vi "Open and Setup CAN Session.vi"(8 "error in":errorcluster, 11 "measurement configuration":T1 {"Baudrate" format="%x"; "FD Baudrate" format="%x"}) -> (0 "error out":errorcluster, 2 "session out":refnum<k21>)   [LabVIEW 2025, in "CAN-LIN Raw Bus Capture.lvclass"]
uses:
  CAN-LIN Raw Bus Capture.lvclass
  Measurement Configuration.ctl
  CAN-LIN Raw Bus Capture UI/Toggle.ctl
  <vilib>/xnet/xnet.llb/XNET Create Session (Frame Input Stream).vi
  CAN-LIN Raw Bus Capture.lvclass/CAN-LIN Raw Bus Capture.ctl
  <resource>/objmgr/xnet.rc
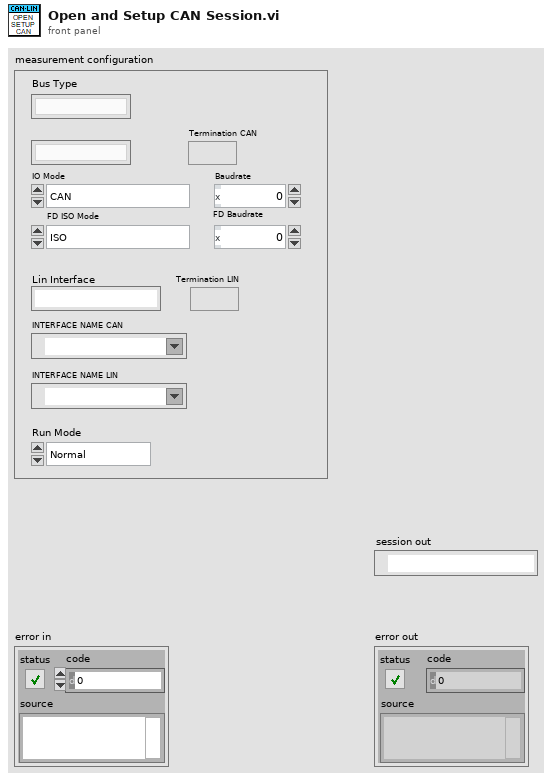
[diagram p1: front panel]
types:
  T1 = typedef "CAN-LIN Raw Bus Capture.lvclass/Measurement Configuration.ctl" = cluster{"Termination CAN":T2, "FD Baudrate":u32, "Baudrate":u32, "FD ISO Mode":enum32{"ISO", "Legacy ISO", "Non-ISO"}, "IO Mode":enum32{"CAN", "CAN FD", "CAN FD + BRS"}, "Termination LIN":T2, "Can Interface":string, "Lin Interface":string, "Bus Type":string, "INTERFACE NAME CAN":refnum<k21>, "INTERFACE NAME LIN":refnum<k21>, "Run Mode":enum32{"Normal", "Subordinate"}}
  T2 = typedef "Toggle.ctl" = bool
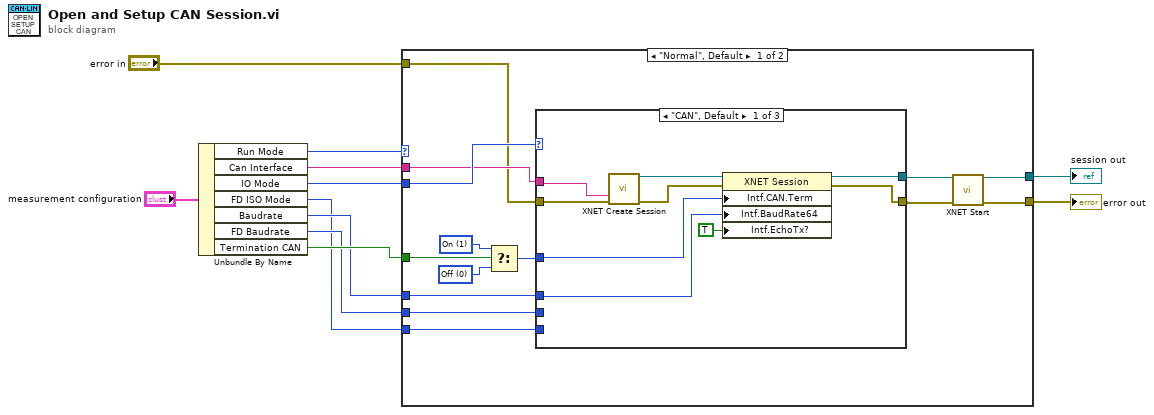
[diagram p0: block diagram]
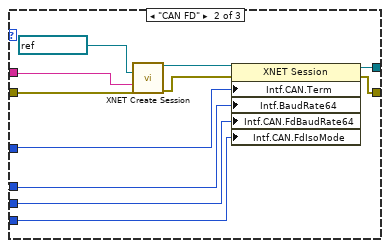
[diagram p2: hidden frame]
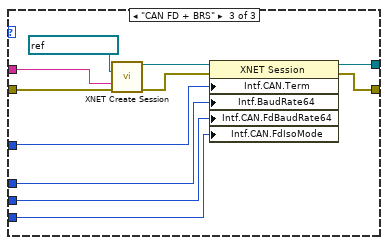
[diagram p3: hidden frame]
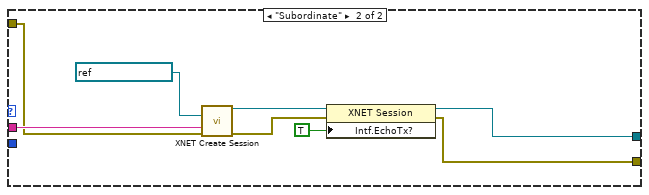
[diagram p4: hidden frame]
diagram:
  n1 = Unbundle By Name("measurement configuration") -> ("Run Mode"=w1:enum32{"Normal", "Subordinate"}, "Can Interface"=w6:string, "IO Mode"=w10:enum32{"CAN", "CAN FD", "CAN FD + BRS"}, "FD ISO Mode"=w7:enum32{"ISO", "Legacy ISO", "Non-ISO"}, "Baudrate"=w9:u32, "FD Baudrate"=w8:u32, "Termination CAN"=w11:T2)
  n2 = case shown="\"Normal\", Default" w1 {
    tunnel: w11 -> [w25 _]
    tunnel: w10 -> [w22 _]
    tunnel: w9 -> [w20 _]
    tunnel: w8 -> [w19 _]
    tunnel: w7 -> [w18 _]
    tunnel: w6 -> [w17 w61]
    tunnel: "error in" -> [w16 w57]
    tunnel: [w13 w58] -> w3
    tunnel: [w12 w59] -> w2
    frame "Normal", Default {
      w23 = u32 1 items=["Off", "On"] ("Interface:CAN:Termination")
      w24 = u32 0 items=["Off", "On"] ("Interface:CAN:Termination")
      n3 = Select(t=w23, s=w25, f=w24) -> (s? t:f=w21:u32)
      n4 = case shown="\"CAN\", Default" w22 {
        tunnel: [w32 w38 w53] -> w15
        tunnel: w17 -> [w29 w42 w49]
        tunnel: w16 -> [w31 w41 w48]
        tunnel: [w30 w37 w46] -> w14
        tunnel: w20 -> [w27 w40 w52]
        tunnel: w19 -> [_ w36 w51]
        tunnel: w18 -> [_ w39 w50]
        tunnel: w21 -> [w28 w35 w47]
        frame "CAN", Default {
          n5 = call-poly <vilib>:"XNET Create Session.vi"("interface"=w29, "error in (no error)"=w31) -> ("session out"=w34:refnum<k21>, "error out"=w33:errorcluster)  [unwired: 12 in]
          n6 = property class="XNET Session"(reference=w34, error in=w33, "Intf.CAN.Term"=w28, "Intf.BaudRate64"=w27, "Intf.EchoTx?"=TRUE ("Interface:Echo Transmit?")) -> (reference out=w32:refnum<k21>, error out=w30:errorcluster)
        }
        frame "CAN FD" {
          n7 = call-poly <vilib>:"XNET Create Session.vi"("cluster (:memory:)"=refnum<k21> ":can_fd:", "interface"=w42, "error in (no error)"=w41) -> ("session out"=w44:refnum<k21>, "error out"=w43:errorcluster)  [unwired: 11 in]
          n8 = property class="XNET Session"(reference=w44, error in=w43, "Intf.CAN.Term"=w35, "Intf.BaudRate64"=w40, "Intf.CAN.FdBaudRate64"=w36, "Intf.CAN.FdIsoMode"=w39) -> (reference out=w38:refnum<k21>, error out=w37:errorcluster)
        }
        frame "CAN FD + BRS" {
          n9 = call-poly <vilib>:"XNET Create Session.vi"("cluster (:memory:)"=refnum<k21> ":can_fd_brs:", "interface"=w49, "error in (no error)"=w48) -> ("session out"=w55:refnum<k21>, "error out"=w54:errorcluster)  [unwired: 11 in]
          n10 = property class="XNET Session"(reference=w55, error in=w54, "Intf.CAN.Term"=w47, "Intf.BaudRate64"=w52, "Intf.CAN.FdBaudRate64"=w51, "Intf.CAN.FdIsoMode"=w50) -> (reference out=w53:refnum<k21>, error out=w46:errorcluster)
        }
      }
      n11 = call <vilib>:"XNET Start.vi"("session in"=w15, "error in (no error)"=w14) -> ("session out"=w12:refnum<k21>, "error out"=w13:errorcluster)  [unwired: 12 in]
    }
    frame "Subordinate" {
      n12 = call-poly <vilib>:"XNET Create Session.vi"("cluster (:memory:)"=refnum<k21> ":subordinate:", "interface"=w61, "error in (no error)"=w57) -> ("session out"=w64:refnum<k21>, "error out"=w63:errorcluster)  [unwired: 11 in]
      n13 = property class="XNET Session"(reference=w64, error in=w63, "Intf.EchoTx?"=TRUE ("Interface:Echo Transmit?")) -> (reference out=w59:refnum<k21>, error out=w58:errorcluster)
    }
  }
  "error out" <- w3
  "session out" <- w2
